vi "SCADA.vi"() -> ()   [LabVIEW 2026]
uses:
  Typedefs/ServoCommand.ctl
  Typedefs/BeltCtrl.ctl
  StateMachine/Globals.vi
panel:
  out "Sort":bool
  out "Classify":bool
  out "Idle":bool
  out "Reject":bool
  out "Purple":bool
  out "Pink":bool
  out "Yellow":bool
  out "Throughput (Obj/min)":dbl
  out "Yellow":dbl
  out "Reject":dbl
  out "Purple":dbl
  out "Pink":dbl
  in  "Conveyer Speed":dbl(knob) min=0.0 max=100.0 scale=0.0..100.0
  in  "Conveyor Belt Control":i16(slide) caption="Slide" scale=0.0..4.0
  in  "Slide Rotation":i16(slide)=3 caption="Slide" scale=0.0..3.0
  in  "Toggle Auto":bool
  in  "Emergency Stop":bool
  out "Live Camera Feed":T1(plugin-control)
  # "State"
  # "Manual / Auto Toggle"
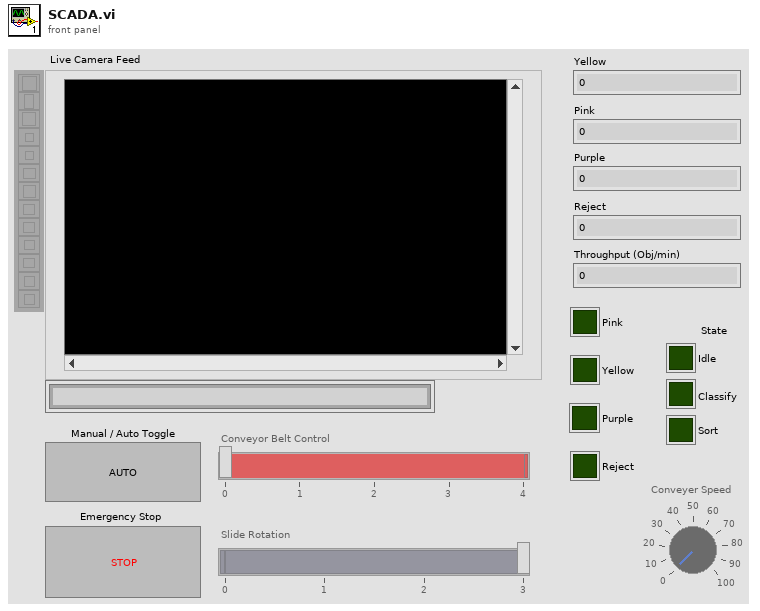
[diagram p1: front panel]
types:
  T1 = typedef "IMAQ Image.ctl" = refnum<image>
  T2 = typedef "BeltCtrl.ctl" = enum16{"Off", "Forward", "Back", "Coast", "Brake", ""}
  T3 = typedef "ServoCommand.ctl" = enum16{"colour 1", "Colour2", "Colour3", "Reject"}
  T4 = enum8{"Enabled", "Disabled", "Disabled and Grayed Out"}
  T5 = typedef "System_State.ctl" = u16
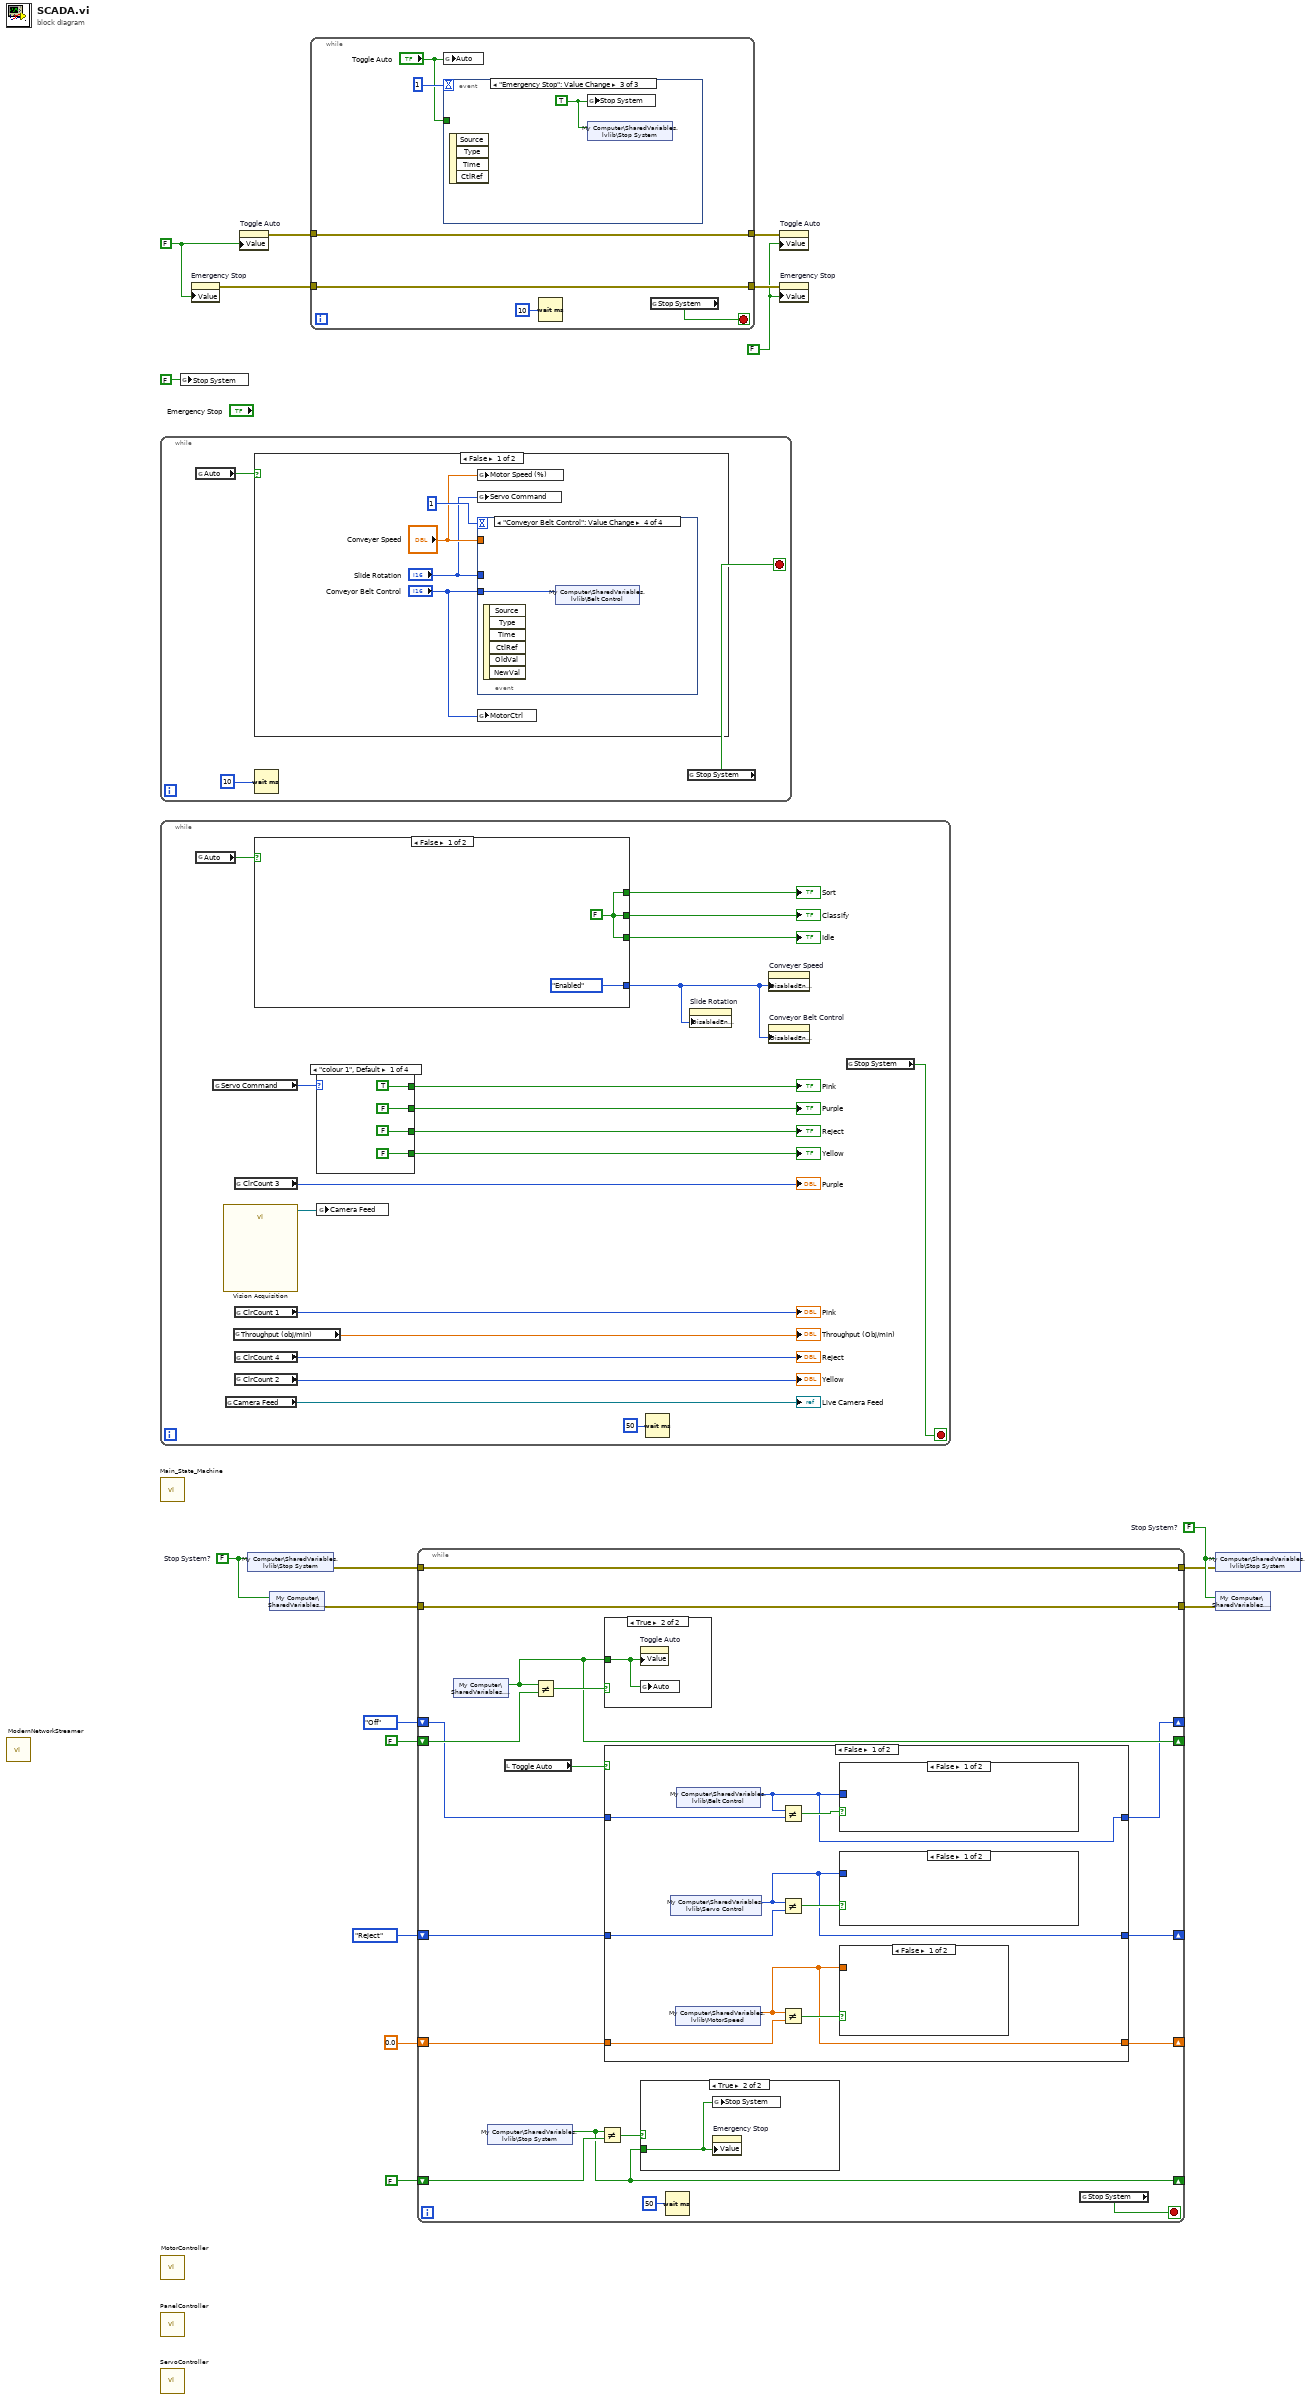
[diagram p0: block diagram]
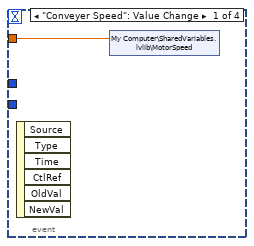
[diagram p2: hidden frame]
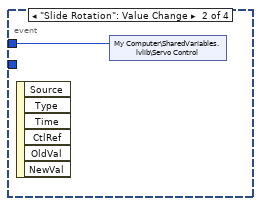
[diagram p3: hidden frame]
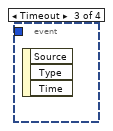
[diagram p4: hidden frame]
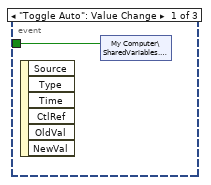
[diagram p6: hidden frame]
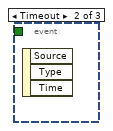
[diagram p7: hidden frame]
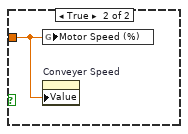
[diagram p8: hidden frame]
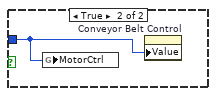
[diagram p9: hidden frame]
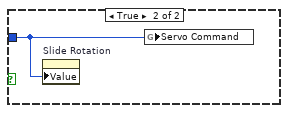
[diagram p10: hidden frame]
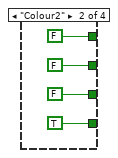
[diagram p14: hidden frame]
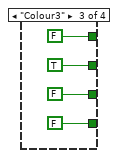
[diagram p15: hidden frame]
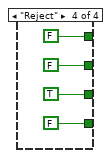
[diagram p16: hidden frame]
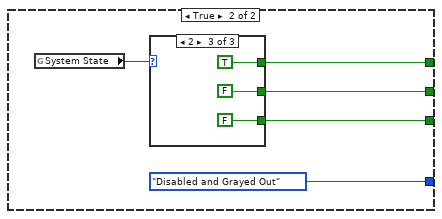
[diagram p17: hidden frame]
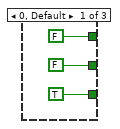
[diagram p18: hidden frame]
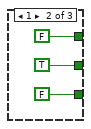
[diagram p19: hidden frame]
diagram:
  w3 = FALSE  # Stop System?
  w7 = FALSE ("Emergency Stop")
  w12 = FALSE ("Emergency Stop")
  w13 = FALSE  # Stop System?
  n1 = call "ModernNetworkStreamer.vi"() -> ()  [unwired: 12 in]
  n2 = while {
    stop <- w20 stop-if-true
    n3 = global read "Globals.vi" "Auto"() -> (w21:bool)
    n4 = case shown="False" w21 {
      frame False {
        n5 = global write "Globals.vi" "Motor Speed (%)"("Conveyer Speed") -> ()
        n6 = global write "Globals.vi" "Servo Command"("Slide Rotation") -> ()
        n7 = event shown="[3] \"Conveyor Belt Control\": Value Change" {
          selector: _ -> [_ _ _ _]
          dyn-events: _ -> [_ _ _ _]
          timeout: 1 -> [_ _ _ _]
          tunnel: "Conveyor Belt Control" -> [_ _ _ w28]
          tunnel: "Conveyer Speed" -> [w26 _ _ _]
          tunnel: "Slide Rotation" -> [_ w27 _ _]
          event "Conveyer Speed": Value Change {
            n8 = event-data() -> ()  [unwired: 1 in, 6 out]
            n9 = shared-variable "My Computer\\SharedVariables.lvlib\\MotorSpeed"(w26) -> ()  [unwired: 1 in, 1 out]
          }
          event "Slide Rotation": Value Change {
            n10 = event-data() -> ()  [unwired: 1 in, 6 out]
            n11 = shared-variable "My Computer\\SharedVariables.lvlib\\Servo Control"(w27) -> ()  [unwired: 1 in, 1 out]
          }
          event Timeout {
            n12 = event-data() -> ()  [unwired: 1 in, 3 out]
          }
          event "Conveyor Belt Control": Value Change {
            n13 = event-data() -> ()  [unwired: 1 in, 6 out]
            n14 = shared-variable "My Computer\\SharedVariables.lvlib\\Belt Control"(w28) -> ()  [unwired: 1 in, 1 out]
          }
        }
        n15 = global write "Globals.vi" "MotorCtrl"("Conveyor Belt Control") -> ()
      }
      frame True {
      }
    }
    n16 = Wait (ms)(milliseconds to wait=u32 10) -> ()  [unwired: 1 out]
    n17 = global read "Globals.vi" "Stop System"() -> (w20:bool)
  }
  n18 = while {
    stop <- w45 stop-if-true
    n19 = global read "Globals.vi" "Auto"() -> (w38:bool)
    n20 = global read "Globals.vi" "Servo Command"() -> (w33:T3)
    n21 = call "Vision Acquisition"() -> ("Image Out"=w29:T1)  [unwired: 25 in, 2 out]
    n22 = global read "Globals.vi" "Camera Feed"() -> (→"Live Camera Feed":T1)
    n23 = global read "Globals.vi" "Throughput (obj/min)"() -> (→"Throughput (Obj/min)":dbl)
    n24 = global read "Globals.vi" "ClrCount 3"() -> (→"Purple":i32)
    n25 = global read "Globals.vi" "ClrCount 1"() -> (→"Pink":i32)
    n26 = global read "Globals.vi" "ClrCount 4"() -> (→"Reject":i32)
    n27 = global read "Globals.vi" "ClrCount 2"() -> (→"Yellow":i32)
    n28 = case shown="False" w38 {
      tunnel: [T4."Enabled" ("Disabled") T4."Disabled and Grayed Out" ("Disabled")] -> w44
      tunnel: [w64 w68] -> w32
      tunnel: [w64 w67] -> w31
      tunnel: [w64 w66] -> w30
      frame False {
        w64 = FALSE
      }
      frame True {
        n29 = global read "Globals.vi" "System State"() -> (w69:T5)
        n30 = case shown="2" w69 {
          tunnel: [TRUE FALSE FALSE] -> w68
          tunnel: [FALSE TRUE FALSE] -> w67
          tunnel: [FALSE FALSE TRUE] -> w66
          frame 0, Default {
          }
          frame 1 {
          }
          frame 2 {
          }
        }
      }
    }
    "Idle" <- w32
    "Classify" <- w31
    "Sort" <- w30
    n31 = case shown="\"colour 1\", Default" w33 {
      tunnel: [FALSE FALSE FALSE TRUE] -> w37
      tunnel: [FALSE FALSE TRUE FALSE] -> w36
      tunnel: [FALSE TRUE FALSE FALSE] -> w35
      tunnel: [TRUE FALSE FALSE FALSE] -> w34
      frame "colour 1", Default {
      }
      frame "Colour2" {
      }
      frame "Colour3" {
      }
      frame "Reject" {
      }
    }
    "Yellow" <- w35
    "Pink" <- w34
    "Purple" <- w36
    "Reject" <- w37
    n32 = global write "Globals.vi" "Camera Feed"(w29) -> ()
    n33 = Wait (ms)(milliseconds to wait=u32 50) -> ()  [unwired: 1 out]
    n34 = property on="Slide Rotation" class="Slide (strict)"("DisabledEnum"=w44) -> ()  [unwired: 2 in, 2 out]
    n35 = property on="Conveyer Speed" class="Knob (strict)"("DisabledEnum"=w44) -> ()  [unwired: 2 in, 2 out]
    n36 = property on="Conveyor Belt Control" class="Slide (strict)"("DisabledEnum"=w44) -> ()  [unwired: 2 in, 2 out]
    n37 = global read "Globals.vi" "Stop System"() -> (w45:bool)
  }
  n38 = call "Main_State_Machine.vi"() -> ()  [unwired: 12 in]
  n39 = call "MotorController.vi"() -> ()  [unwired: 11 in]
  n40 = call "PanelController.vi"() -> ()  [unwired: 12 in]
  n41 = call "ServoController.vi"() -> ()  [unwired: 12 in]
  n42 = global write "Globals.vi" "Stop System"(FALSE ("Stop System")) -> ()
  n43 = property on="Emergency Stop" class="Bool (strict)"("Value"=w12) -> (error out=w11:errorcluster)  [unwired: 2 in, 1 out]
  n44 = property on="Toggle Auto" class="Bool (strict)"("Value"=w12) -> (error out=w10:errorcluster)  [unwired: 2 in, 1 out]
  n45 = shared-variable "My Computer\\SharedVariables.lvlib\\Stop System"(w13) -> (error out=w5:errorcluster)  [unwired: 1 in]
  n46 = shared-variable "My Computer\\SharedVariables.lvlib\\Auto"(w13) -> (error out=w4:errorcluster)  [unwired: 1 in]
  n47 = while {
    tunnel: w11 -> [w81]
    tunnel: w10 -> [w82]
    tunnel: [w82] -> w9
    tunnel: [w81] -> w8
    stop <- w85 stop-if-true
    n48 = global write "Globals.vi" "Auto"("Toggle Auto") -> ()
    n49 = event shown="[2] \"Emergency Stop\": Value Change" {
      selector: _ -> [_ _ _]
      dyn-events: _ -> [_ _ _]
      timeout: 1 -> [_ _ _]
      tunnel: "Toggle Auto" -> [w86 _ _]
      event "Toggle Auto": Value Change {
        n50 = event-data() -> ()  [unwired: 1 in, 6 out]
        n51 = shared-variable "My Computer\\SharedVariables.lvlib\\Auto"(w86) -> ()  [unwired: 1 in, 1 out]
      }
      event Timeout {
        n52 = event-data() -> ()  [unwired: 1 in, 3 out]
      }
      event "Emergency Stop": Value Change {
        w87 = TRUE
        n53 = event-data() -> ()  [unwired: 1 in, 4 out]
        n54 = global write "Globals.vi" "Stop System"(w87) -> ()
        n55 = shared-variable "My Computer\\SharedVariables.lvlib\\Stop System"(w87) -> ()  [unwired: 1 in, 1 out]
      }
    }
    n56 = Wait (ms)(milliseconds to wait=u32 10) -> ()  [unwired: 1 out]
    n57 = global read "Globals.vi" "Stop System"() -> (w85:bool)
  }
  n58 = while {
    shift-right: [w90] -> _
    shift-left: FALSE ("Boolean") -> [w99]
    shift-right: [w98] -> _
    shift-left: FALSE ("Boolean") -> [w97]
    shift-right: [w96] -> _
    shift-left: 0.0 ("Double") -> [w95]
    shift-right: [w94] -> _
    shift-left: ServoCommand."Reject" ("Servo Command") -> [w92]
    shift-right: [w93] -> _
    shift-left: BeltCtrl."Off" ("BeltCtrl") -> [w91]
    tunnel: w5 -> [w89]
    tunnel: w4 -> [w88]
    tunnel: [w89] -> w2
    tunnel: [w88] -> w1
    stop <- w102 stop-if-true
    n59 = shared-variable "My Computer\\SharedVariables.lvlib\\Auto"() -> (w98:bool)  [unwired: 1 in, 1 out]
    n60 = shared-variable "My Computer\\SharedVariables.lvlib\\Stop System"() -> (w90:bool)  [unwired: 1 in, 1 out]
    n61 = local read "Toggle Auto"() -> (w101:bool)
    n62 = Not Equal?(x=w98, y=w97) -> (x != y?=w104:bool)
    n63 = Not Equal?(x=w90, y=w99) -> (x != y?=w103:bool)
    n64 = case shown="True" w104 {
      tunnel: w98 -> [_ w121]
      frame False {
      }
      frame True {
        n65 = property on="Toggle Auto" class="Bool (strict)"("Value"=w121) -> ()  [unwired: 2 in, 2 out]
        n66 = global write "Globals.vi" "Auto"(w121) -> ()
      }
    }
    n67 = case shown="False" w101 {
      tunnel: [w110 w119] -> w96
      tunnel: w95 -> [w109 w119]
      tunnel: [w108 w118] -> w94
      tunnel: [w107 w117] -> w93
      tunnel: w92 -> [w106 w118]
      tunnel: w91 -> [w105 w117]
      frame False {
        n68 = shared-variable "My Computer\\SharedVariables.lvlib\\Servo Control"() -> (w108:T3)  [unwired: 1 in, 1 out]
        n69 = shared-variable "My Computer\\SharedVariables.lvlib\\MotorSpeed"() -> (w110:dbl)  [unwired: 1 in, 1 out]
        n70 = shared-variable "My Computer\\SharedVariables.lvlib\\Belt Control"() -> (w107:T2)  [unwired: 1 in, 1 out]
        n71 = Not Equal?(x=w107, y=w105) -> (x != y?=w112:bool)
        n72 = Not Equal?(x=w108, y=w106) -> (x != y?=w113:bool)
        n73 = Not Equal?(x=w110, y=w109) -> (x != y?=w111:bool)
        n74 = case shown="False" w112 {
          tunnel: w107 -> [_ w115]
          frame False {
          }
          frame True {
            n75 = global write "Globals.vi" "MotorCtrl"(w115) -> ()
            n76 = property on="Conveyor Belt Control" class="Slide (strict)"("Value"=w115) -> ()  [unwired: 2 in, 2 out]
          }
        }
        n77 = case shown="False" w113 {
          tunnel: w108 -> [_ w116]
          frame False {
          }
          frame True {
            n78 = property on="Slide Rotation" class="Slide (strict)"("Value"=w116) -> ()  [unwired: 2 in, 2 out]
            n79 = global write "Globals.vi" "Servo Command"(w116) -> ()
          }
        }
        n80 = case shown="False" w111 {
          tunnel: w110 -> [_ w114]
          frame False {
          }
          frame True {
            n81 = global write "Globals.vi" "Motor Speed (%)"(w114) -> ()
            n82 = property on="Conveyer Speed" class="Knob (strict)"("Value"=w114) -> ()  [unwired: 2 in, 2 out]
          }
        }
      }
      frame True {
      }
    }
    n83 = case shown="True" w103 {
      tunnel: w90 -> [_ w120]
      frame False {
      }
      frame True {
        n84 = global write "Globals.vi" "Stop System"(w120) -> ()
        n85 = property on="Emergency Stop" class="Bool (strict)"("Value"=w120) -> ()  [unwired: 2 in, 2 out]
      }
    }
    n86 = Wait (ms)(milliseconds to wait=u32 50) -> ()  [unwired: 1 out]
    n87 = global read "Globals.vi" "Stop System"() -> (w102:bool)
  }
  n88 = property on="Toggle Auto" class="Bool (strict)"(error in=w9, "Value"=w7) -> ()  [unwired: 1 in, 2 out]
  n89 = property on="Emergency Stop" class="Bool (strict)"(error in=w8, "Value"=w7) -> ()  [unwired: 1 in, 2 out]
  n90 = shared-variable "My Computer\\SharedVariables.lvlib\\Stop System"(w3, error in=w2) -> ()  [unwired: 1 out]
  n91 = shared-variable "My Computer\\SharedVariables.lvlib\\Auto"(w3, error in=w1) -> ()  [unwired: 1 out]
